vi "MQTT Session - Keep Alive.vi"(0 "mqtt ref in":T1, 11 "error in":errorcluster) -> (4 "mqtt ref out":T1, 8 "Version":u8, 15 "error out":errorcluster)   [LabVIEW 2019, in "KoRE-MQTT.lvlib"]
doc: "Sends a PINGREQ message to the server if the keep alive timer has passed (i.e. if half the time of the keep alive time has passed) and return the sessions MQTT version (conveniently placed!)\n\nAuthor: Kåre Langedrag\n\nCopyright (c) 2025 KoRElibs.com\nSPDX-License-Identifier: EUPL-1.2\n\nThis VI is licensed under the European Union Public License (EUPL) Version 1.2. You may use this VI unmodified in proprietary works. If you distribute a modified version of this file, the modified file must be released under the EUPL-1.2. Full license: https://joinup.ec.europa.eu/asset/eupl/eupl/1.2/"
uses:
  KoRE-MQTT.lvlib
  Public/TypeDefs/MQTT Client Session.ctl
  TypeDefs/MQTT Client Session - Data Value Reference.ctl
  Public/TypeDefs/MQTT Client Session - Data.ctl
  Public/TypeDefs/MQTT Property - Will.ctl
  Public/TypeDefs/MQTT Property - CONNECT.ctl
  TypeDefs/MQTT Subscription - Info.ctl
  TypeDefs/MQTT Packet - Type.ctl
  MQTT Session - Get TCP Info.vi
  MQTT Session - Reset Keep Alive Timer.vi
  MQTT Data Stream - Write Packet.vi
  MQTT Data - Encode Varint.vi
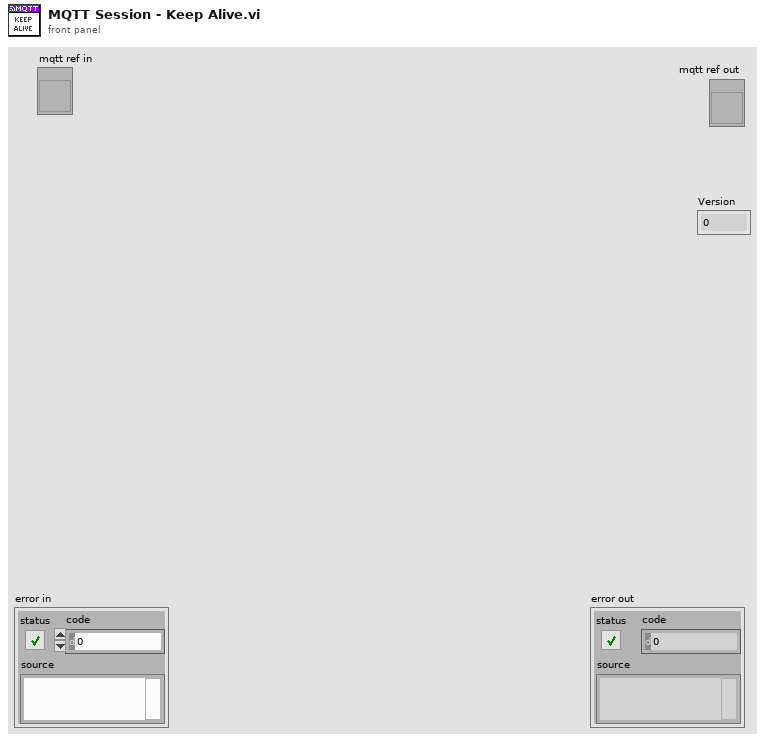
[diagram p1: front panel]
types:
  T1 = typedef "KoRE-MQTT.lvlib/MQTT Client Session.ctl" = refnum<vi>
  T2 = typedef "KoRE-MQTT.lvlib/MQTT Client Session - Data Value Reference.ctl" = refnum<data-value>
  T3 = typedef "KoRE-MQTT.lvlib/MQTT Packet - Type.ctl" = enum32{"Reserved", "CONNECT", "CONNACK", "PUBLISH", "PUBACK", "PUBREC", "PUBREL", "PUBCOMP", "SUBSCRIBE", "SUBACK", "UNSUBSCRIBE", "UNSUBACK", "PINGREQ", "PINGRESP", "DISCONNECT", "AUTH"}
  T4 = typedef "KoRE-MQTT.lvlib/MQTT Client Session - Data.ctl" = cluster{"TCP ref":refnum<k5>, "Next Packet Id":u16, "Version":u8, "Host":string, "Port":u16, "Ping Delta":u32, "Username":string, "Password":string, "Will QoS":u8, "Will Retain":bool, "Will Topic":string, "Will Payload":string, "TCP Timeout":i32, "Semaphore":T5, "In-Flight Messages":variant, "Close":bool, "Last Send":u32, "Keep Alive":u16, "Last Ping RTT":u32, "Last Ping":u32, "Will Properties":T6[], "Session Expiry Interval":u32, "Maximum QoS":u8, "Retain Available":bool, "Server Maximum Packet Size":u32, "Client Identifier":string, "Server Topic Alias Maximum":u16, "Wildcard Subscription Available":bool, "Subscription Identifier Available":bool, "Shared Subscription Available":bool, "Connect Properties":T7[], "Client Maximum Packet Size":u32, "Client Topic Alias Maximum":u16, "Server Receive Maximum":u16, "Client Receive Maximum":u16, "TLS cfg":refnum<k36>, "Subscriptions":T8[]}
  T5 = typedef "Semaphore RefNum" = refnum<k1>
  T6 = typedef "KoRE-MQTT.lvlib/MQTT Property - Will.ctl" = cluster{"Property":u8, "Value":string}
  T7 = typedef "KoRE-MQTT.lvlib/MQTT Property - CONNECT.ctl" = cluster{"Property":u8, "Value":string}
  T8 = typedef "KoRE-MQTT.lvlib/MQTT Subscription - Info.ctl" = cluster{"Packet Id":u16, "Index":u16, "Identifier":u32, "QoS":u8, "Topic Filter":string, "Reason Code":u8, "Reason String":string, "Granted":bool}
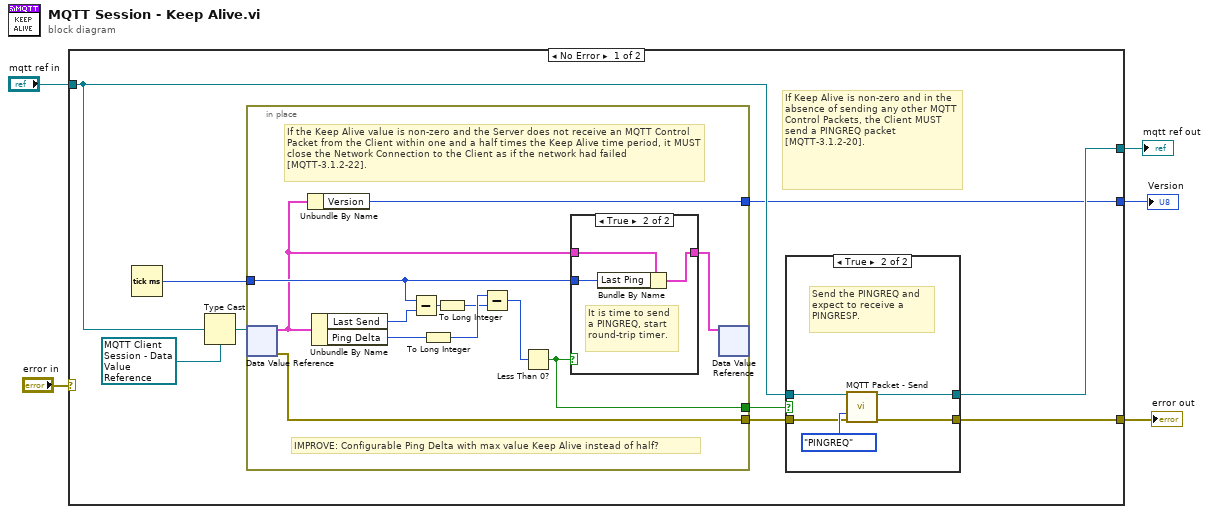
[diagram p0: block diagram]
diagram:
  n1 = case shown="No Error" "error in" {
    selector: "error in" -> [_ w39]
    tunnel: "mqtt ref in" -> [w12 w38]
    tunnel: [w10 w39] -> w4
    tunnel: [w8 w38] -> w2
    tunnel: [w6 _] -> w1
    frame No Error {
      # "If Keep Alive is non-zero and in the absence of sending any other MQTT Control Packets, the Client MUST send a PINGREQ packet [MQTT-3.1.2-20]."
      n2 = Tick Count (ms)() -> (millisecond timer value=w7:u32)
      n3 = Type Cast(type=T2 refnum ("data value reference"), x=w12) -> (*(type *) &x=w13:T2)
      n4 = in-place {
        in-place-border: [w26] -> w11
        in-place-border: [w17] -> w9
        in-place-border: w7 -> [w18]
        in-place-border: [w15] -> w6
        # "IMPROVE: Configurable Ping Delta with max value Keep Alive instead of half?"
        # "If the Keep Alive value is non-zero and the Server does not receive an MQTT Control Packet from the Client within one and a half times the Keep Alive time period, it MUST close the Network Connection to the Client as if the network had failed [MQTT-3.1.2-22]."
        n5 = in-place-dvr #1(w13) -> (w16:T4, w26:errorcluster)
        n6 = Unbundle By Name(w16) -> ("Version"=w15:u8)
        n7 = Unbundle By Name(w16) -> ("Last Send"=w25:u32, "Ping Delta"=w24:u32)
        n8 = Subtract(x=w18, y=w25) -> (x-y=w23:u32)
        n9 = To Long Integer(number=w24) -> (32bit integer=w21:i32)
        n10 = To Long Integer(number=w23) -> (32bit integer=w20:i32)
        n11 = Subtract(x=w21, y=w20) -> (x-y=w22:i32)
        n12 = Less Than 0?(x=w22) -> (x < 0?=w17:bool)
        n13 = case shown="True" w17 {
          tunnel: w16 -> [w27 w30]
          tunnel: [w27 w29] -> w19
          tunnel: w18 -> [_ w28]
          frame False {
          }
          frame True {
            # "It is time to send\na PINGREQ, start\nround-trip timer."
            n14 = Bundle By Name(cluster=w30, "Last Ping"=w28) -> (w29:T4)
          }
        }
        n15 = in-place-dvr #1(w19) -> ()  [unwired: 2 out]
      }
      n16 = case shown="True" w9 {
        tunnel: w12 -> [w31 w37]
        tunnel: w11 -> [w32 w35]
        tunnel: [w32 w33] -> w10
        tunnel: [w31 w34] -> w8
        frame False {
        }
        frame True {
          # "Send the PINGREQ and\nexpect to receive a \nPINGRESP."
          n17 = call "MQTT Packet - Send.vi"("mqtt ref in"=w37, "MessageType"=MQTT_Packet_-_Type."PINGREQ", "error in (no error)"=w35) -> ("mqtt ref out"=w34:T1, "error out"=w33:errorcluster)  [unwired: 10 in, 1 out]
        }
      }
    }
    frame Error {
    }
  }
  "error out" <- w4
  "Version" <- w1
  "mqtt ref out" <- w2
